vi "Test_Case_editer.vi"(3 "Edit Button":bool, 11 "Table Control 5":string[][](table)) -> ()   [LabVIEW 2021]
uses:
  <vilib>/Utility/file.llb/Read Delimited Spreadsheet (string).vi
  <vilib>/Utility/file.llb/Write Delimited Spreadsheet (string).vi
panel:
  in  "error in":errorcluster
  out "Table Control 6":string[][](array[string])
  out "Multicolumn Listbox 3":i32(listbox)
  in  "Multicolumn Listbox 2":i32(listbox)
  out "all rows":string[][](array[string])
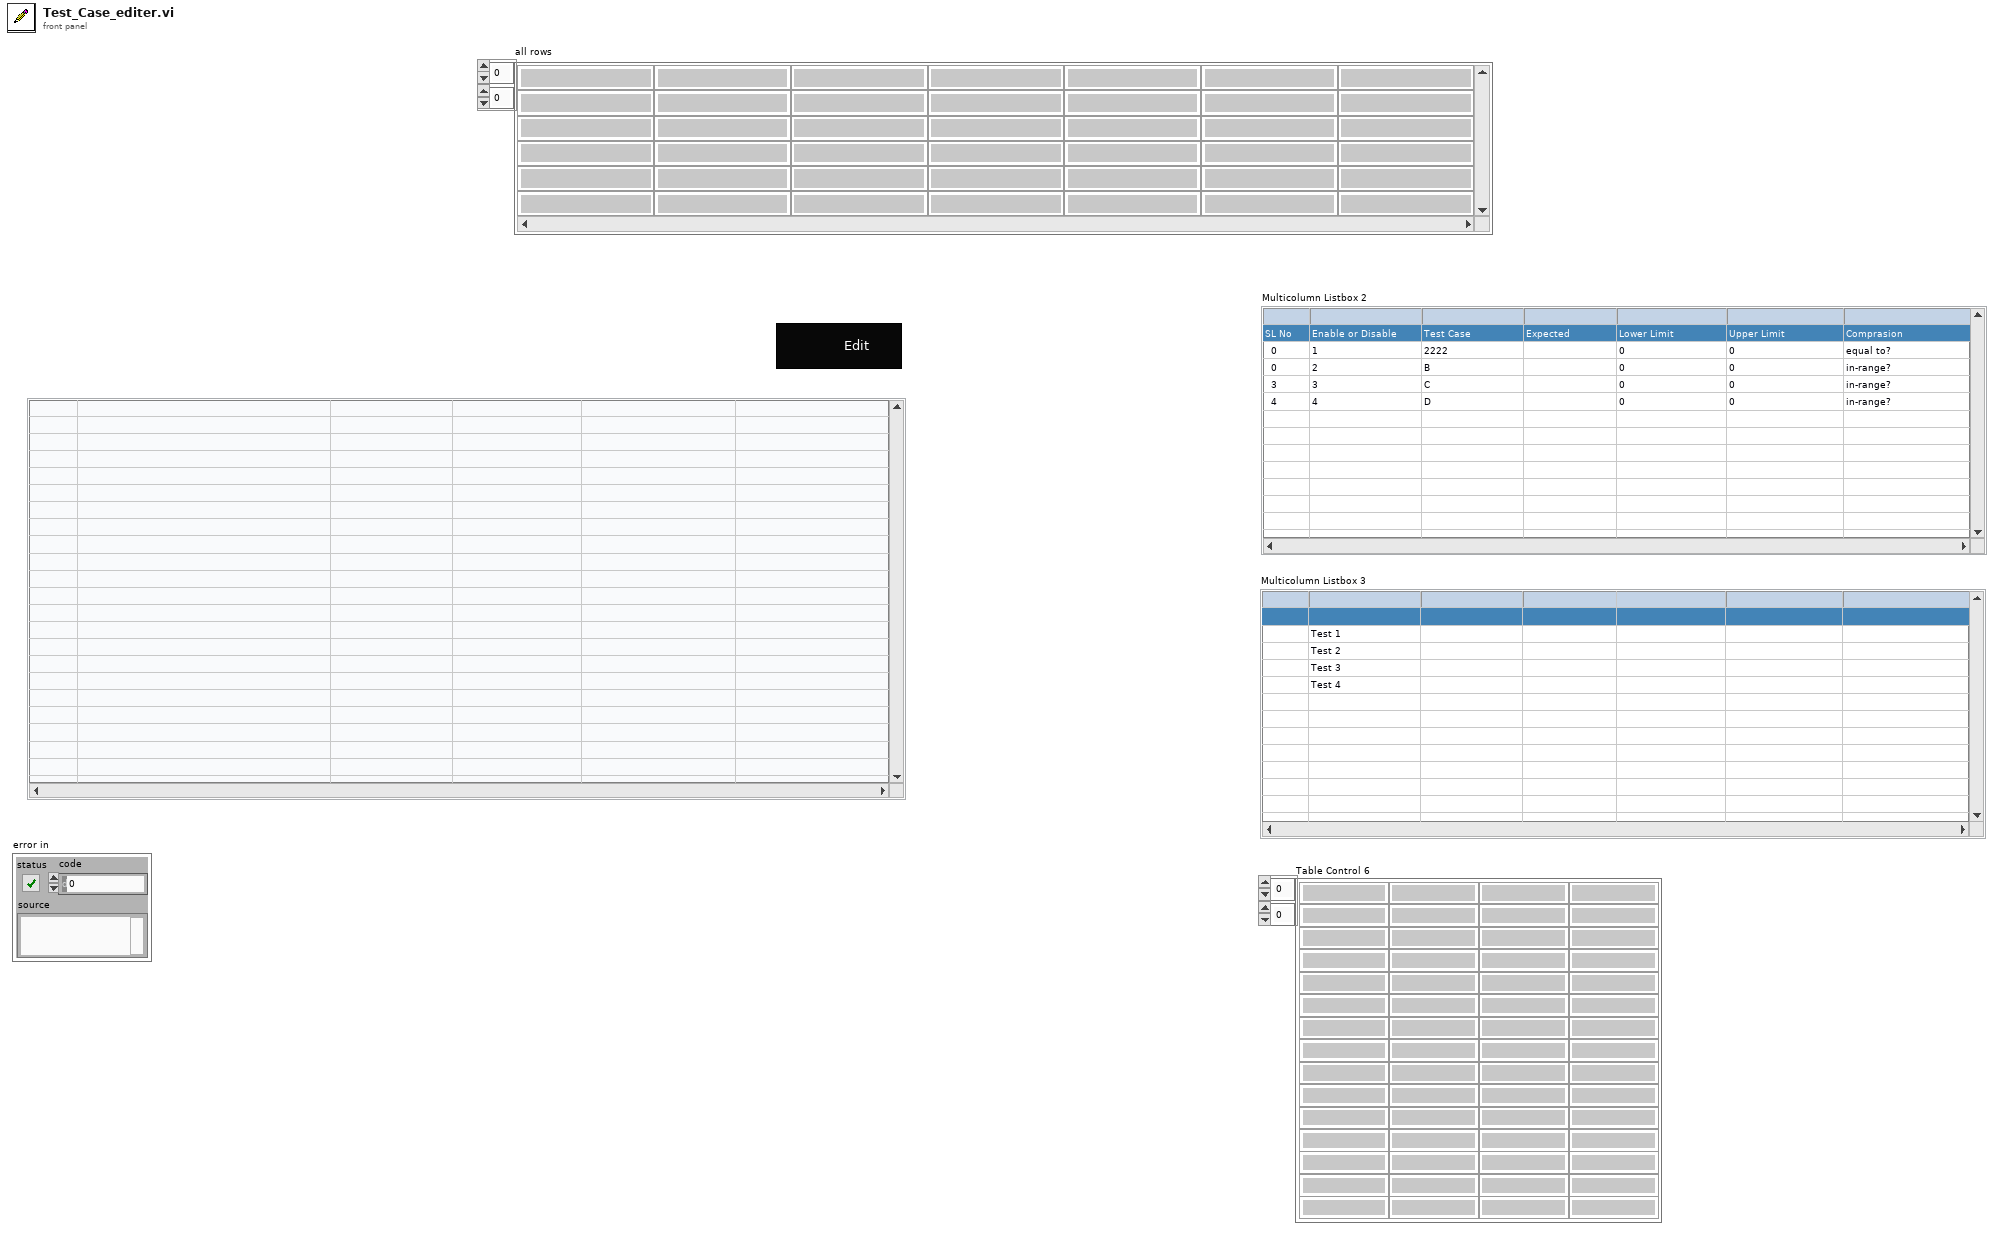
[diagram p1: front panel]
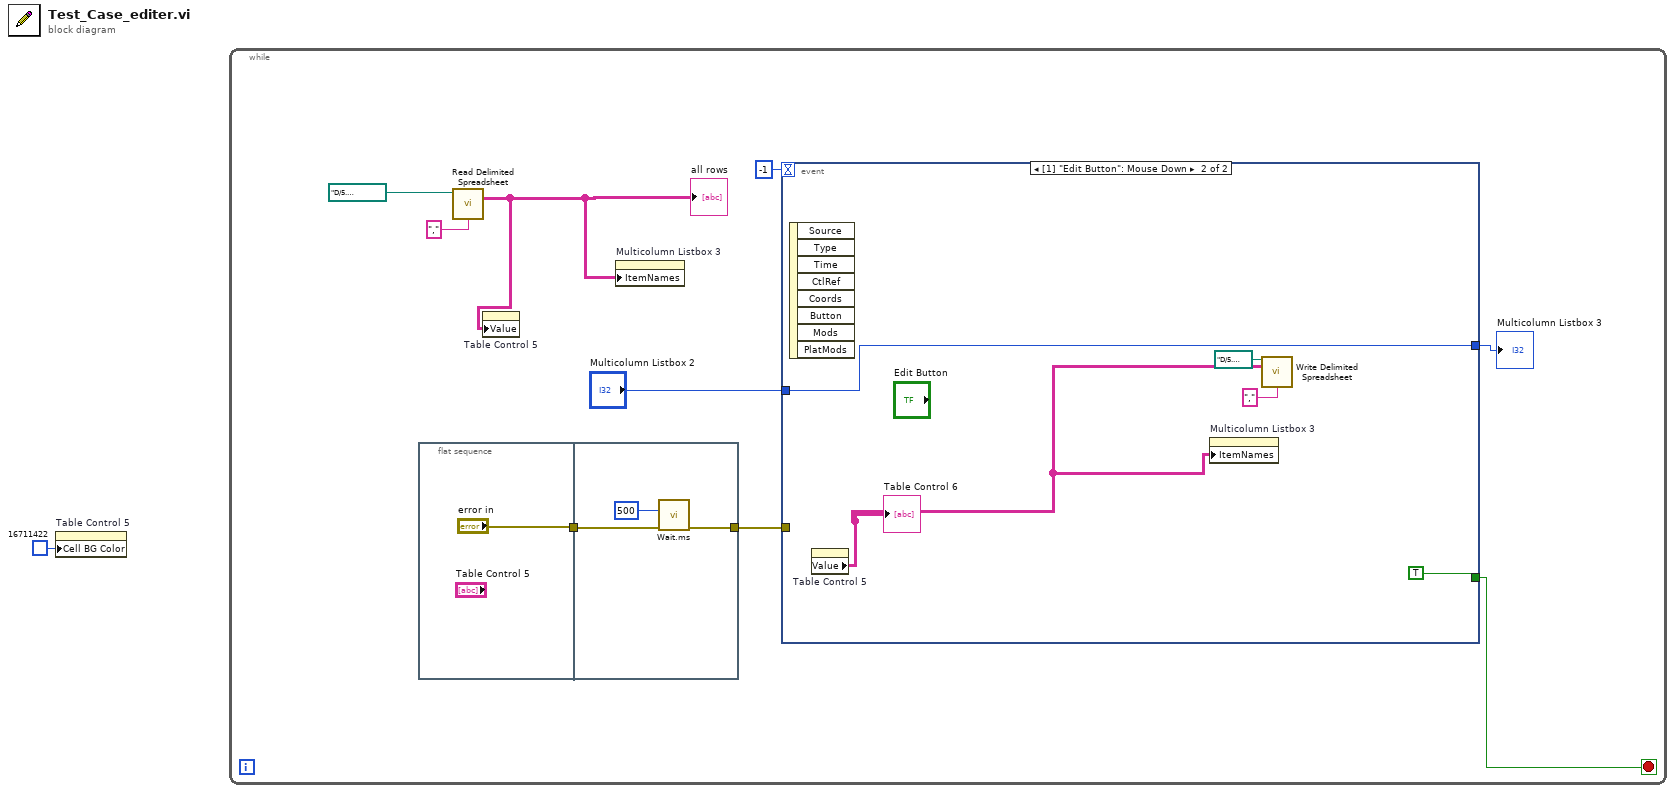
[diagram p0: block diagram]
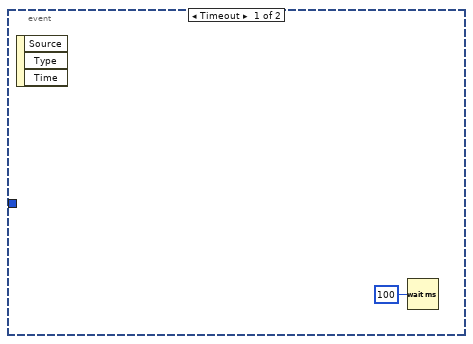
[diagram p2: hidden frame]
diagram:
  n1 = property on="Table Control 5" class="Tbl (strict)"("Cell BG Color"=u32 16711422 ("Active Cell:Cell Background Color")) -> ()  [unwired: 2 in, 2 out]
  n2 = while {
    stop <- w2 stop-if-true
    n3 = flat-sequence {
      tunnel: ["error in"] -> w10
      tunnel: w10 -> [w13]
      tunnel: [w12] -> w3
      frame #0 {
      }
      frame #1 {
        n4 = call "Wait.ms.vi"("error in"=w13, "milliseconds to wait"=u32 500) -> ("error out"=w12:errorcluster)  [unwired: 9 in]
      }
    }
    n5 = call-poly <vilib>:"Read Delimited Spreadsheet.vi"("file path (dialog if empty)"=path "D:/5.ACTIVITIES/LabVIEW_State_Machine_Template/LabVIEW_State_Machine_Template/LabVIEW_State_Machine_Template/Project_Template/Template/Data/Test_Flow.csv", "delimiter (\\t)"="," ("delimiter (\\t)")) -> ("all rows"=w4:string[][])  [unwired: 8 in, 5 out]
    "all rows" <- w4
    n6 = property on="Table Control 5" class="Tbl (strict)"("Value"=w4) -> ()  [unwired: 2 in, 2 out]
    n7 = property on="Multicolumn Listbox 3" class="MCListbox (strict)"("ItemNames"=w4) -> ()  [unwired: 2 in, 2 out]
    n8 = event shown="[1] \"Edit Button\": Mouse Down" {
      selector: _ -> [_ _]
      dyn-events: _ -> [_ _]
      timeout: -1 -> [_ _]
      tunnel: [_ w17] -> w6
      tunnel: [_ TRUE] -> w2
      tunnel: "Multicolumn Listbox 2" -> [_ w17]
      tunnel: w3 -> [_ _]
      event Timeout {
        n9 = event-data() -> ()  [unwired: 1 in, 3 out]
        n10 = Wait (ms)(milliseconds to wait=u32 100) -> ()  [unwired: 1 out]
      }
      event "Edit Button": Mouse Down {
        n11 = event-data() -> ()  [unwired: 1 in, 8 out]
        n12 = property on="Table Control 5" class="Tbl (strict)"() -> ("Value"=w16:string[][])  [unwired: 2 in, 2 out]
        "Table Control 6" <- w16
        n13 = property on="Multicolumn Listbox 3" class="MCListbox (strict)"("ItemNames"=w16) -> ()  [unwired: 2 in, 2 out]
        n14 = call-poly <vilib>:"Write Delimited Spreadsheet.vi"("file path (dialog if empty)"=path "D:/5.ACTIVITIES/LabVIEW_State_Machine_Template/LabVIEW_State_Machine_Template/LabVIEW_State_Machine_Template/Project_Template/Template/Data/Test_Flow.csv", "2D data"=w16, "delimiter (\\t)"="," ("delimiter (\\t)")) -> ()  [unwired: 11 in, 2 out]
      }
    }
    "Multicolumn Listbox 3" <- w6
  }
